vi "Add Rx Label.vi"(6 "create channels":T1, 7 "label (Display)":u32, 8 "error in":errorcluster, 9 "SDI value":T3=-1 items=["All"=-1, "0 (b00)"=0, "1 (b01)"=1, "2 (b10)"=2, "3 (b11)"=3], 10 "label (Dec)":u32, 11 "port in":T2 format="%.0x") -> (0 "error out":errorcluster, 2 "label":T2 format="%.0x", 3 "port out":T2 format="%.0x")   [LabVIEW 2020, in "Ballard ARINC 429 Scripting.lvlib"]
doc: "Adds an Rx label to the specified incoming (Rx) port. Returns the newly added <b>label</b> reference."
uses:
  Ballard ARINC 429 Scripting.lvlib
  Constants.vi
  ARINC 429/ARINC 429 Scripting.lvlib
  <vilib>/NI VeriStand/Custom Device API/Custom Device Channel Type.ctl
  <vilib>/NI VeriStand/Custom Device API/Custom Device API.lvlib
  <vilib>/NI VeriStand/Custom Device API/Custom Device Channel.ctl
  Shared/Label Properties.ctl
  Shared/Label.ctl
  Import/ARINC 429 Import.lvlib
  ARINC 429/Constants.vi
  <vilib>/NI VeriStand/Custom Device API/Custom Device Item Ref.ctl
  <vilib>/NI VeriStand/Custom Device Offline API/Custom Device Offline API.lvlib
  Shared/SDI.ctl
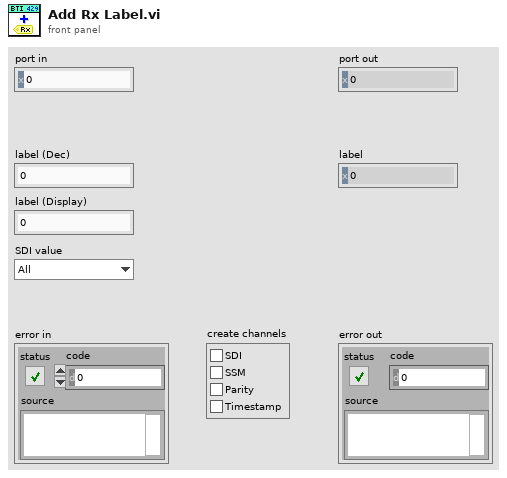
[diagram p1: front panel]
types:
  T1 = cluster{"SDI":bool, "SSM":bool, "Parity":bool, "Timestamp":bool}
  T2 = typedef "Custom Device API.lvlib/Custom Device Item Ref.ctl" = u64
  T3 = typedef "SDI.ctl" = i32
  T4 = typedef "Direction.ctl" = enum16{"Rx", "Tx"}
  T5 = typedef "Custom Device API.lvlib/Custom Device Channel.ctl" = cluster{"Type":T6, "Units":string, "Default Value":dbl, "Faultable":bool, "Scalable":bool}
  T6 = typedef "Custom Device API.lvlib/Custom Device Channel Type.ctl" = enum16{"Input", "Output"}
  T7 = typedef "Label Properties.ctl" = cluster{"label (Dec)":T8, "SDI value":u8, "SDI enabled":bool}
  T8 = typedef "Label.ctl" = u8
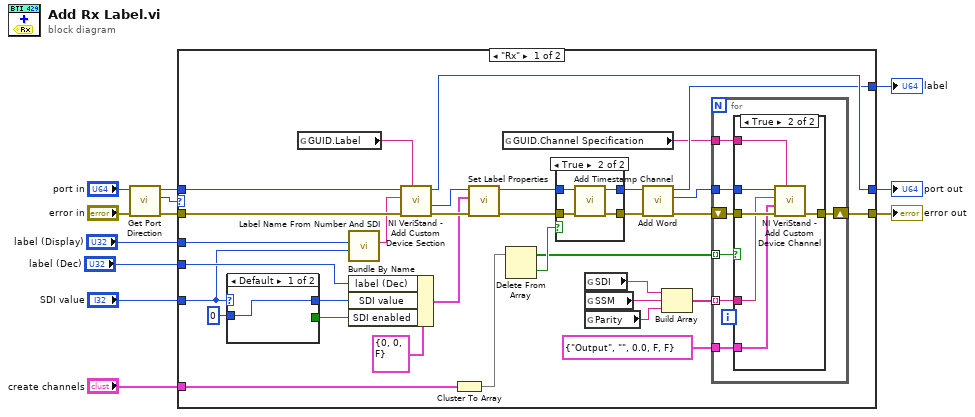
[diagram p0: block diagram]
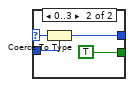
[diagram p4: hidden frame]
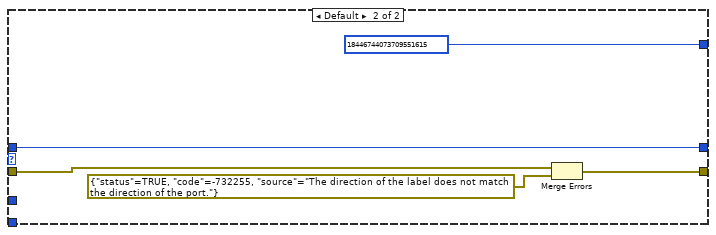
[diagram p5: hidden frame]
diagram:
  n1 = call "Get Port Direction.vi"("error in"="error in", "port ref in"="port in") -> ("error out"=w9:errorcluster, "direction"=w2:T4, "port ref out"=w10:T2)  [unwired: 7 in]
  n2 = case shown="\"Rx\"" w2 {
    tunnel: w10 -> [w37 w75]
    tunnel: w9 -> [w36 w73]
    tunnel: [w33 w75] -> w8
    tunnel: "label (Dec)" -> [w30 _]
    tunnel: "SDI value" -> [w28 _]
    tunnel: "create channels" -> [w27 _]
    tunnel: [w24 T2 18446744073709551615 ("label ref out")] -> w4
    tunnel: [w22 w72] -> w3
    tunnel: "label (Display)" -> [w13 _]
    frame "Rx" {
      n3 = case shown="Default" w28 {
        selector: w28 -> [_ w70]
        tunnel: [w66 w67] -> w29
        tunnel: u8 0 ("SDI value") -> [w66 w69]
        tunnel: [_ TRUE] -> w34
        frame Default {
        }
        frame 0..3 {
          n4 = Coerce To Type(0:w70, 1:w69) -> (2:w67:u8)
        }
      }
      n5 = global read "Constants.vi" "GUID.Label"() -> (w40:string)
      n6 = call "Label Name From Number And SDI.vi"("SDI value"=w28, "label (Display)"=w13) -> ("label name"=w31:string)  [unwired: 9 in]
      n7 = Bundle By Name(cluster=T7 {"label (Dec)"=0, "SDI value"=0, "SDI enabled"=FALSE} ("label properties"), "label (Dec)"=w30, "SDI value"=w29, "SDI enabled"=w34) -> (w38:T7)
      n8 = call <vilib>:"NI VeriStand - Add Custom Device Section.vi"("GUID (Default Section)"=w40, "error in (no error)"=w36, "Section Name"=w31, "Parent Ref in"=w37) -> ("error out"=w42:errorcluster, "Section Ptr"=w41:T2, "Parent Ref out"=w33:T2)  [unwired: 4 in, 1 out]
      n9 = Cluster To Array(cluster=w27) -> (array=w26:bool[])
      n10 = call "Set Label Properties.vi"("error in"=w42, "label properties"=w38, "label ref"=w41) -> ("error out"=w43:errorcluster, "label ref out"=w32:T2)  [unwired: 7 in]
      n11 = global read "Constants.vi" "GUID.Channel Specification"() -> (w19:string)
      n12 = Delete From Array(array=w26) -> (deleted portion=w25:bool, array with subset deleted=w21:bool[])  [unwired: 2 in]
      n13 = case shown="True" w25 {
        tunnel: [w61 w65] -> w45
        tunnel: [w60 w64] -> w44
        tunnel: w43 -> [w60 w63]
        tunnel: w32 -> [w61 w62]
        frame False {
        }
        frame True {
          n14 = call "Add Timestamp Channel.vi"("error in"=w63, "label ref"=w62) -> ("error out"=w64:errorcluster, "label ref out"=w65:T2)  [unwired: 8 in]
        }
      }
      n15 = global read "Constants.vi" "SDI"() -> (w16:string)
      n16 = global read "Constants.vi" "SSM"() -> (w17:string)
      n17 = global read "Constants.vi" "Parity"() -> (w15:string)
      n18 = call "Add Word.vi"("error in"=w44, "label ref"=w45) -> ("error out"=w23:errorcluster, "word ref"=w20:T2, "label ref out"=w24:T2)  [unwired: 6 in, 1 out]
      n19 = Build Array(w16, w17, w15) -> (w14:string[])
      n20 = for {
        shift-right: [w51] -> w22
        shift-left: w23 -> [w50]
        tunnel: w21 -> [w52] mode=indexing
        tunnel: w20 -> [w49]
        tunnel: w19 -> [w48]
        tunnel: T5 {"Type"=enum."Output", "Units"="", "Default Value"=0.0, "Faultable"=FALSE, "Scalable"=FALSE} ("Channel") -> [w47]
        tunnel: w14 -> [w46] mode=indexing
        n21 = case shown="True" w52 {
          tunnel: [w53 w59] -> w51
          tunnel: w50 -> [w53 w58]
          tunnel: w49 -> [_ w55]
          tunnel: w48 -> [_ w57]
          tunnel: w47 -> [_ w56]
          tunnel: w46 -> [_ w54]
          frame False {
          }
          frame True {
            n22 = call <vilib>:"NI VeriStand - Add Custom Device Channel.vi"("GUID (Default Channel)"=w57, "error in (no error)"=w58, "Channel"=w56, "Channel Name"=w54, "Parent Ref in"=w55) -> ("error out"=w59:errorcluster)  [unwired: 3 in, 3 out]
          }
        }
      }
    }
    frame Default {
      n23 = Merge Errors(w73, errorcluster {"status"=TRUE, "code"=-732255, "source"="The direction of the label does not match the direction of the port."} ("error in")) -> (w72:errorcluster)
    }
  }
  "label" <- w4
  "error out" <- w3
  "port out" <- w8
